vi "50-2.vi"() -> ()   [LabVIEW 2025]
uses:
  <vilib>/Platform/TimedLoop/XDataNode/timing_clust.ctl
  <vilib>/Platform/TimedLoop/XDataNode/nitl_modes.ctl
  <vilib>/Platform/TimedLoop/XDataNode/wakeup.ctl
  <vilib>/eio/utilities/niEioResolveVilibRelativePath.vi
  <vilib>/rvi/interface/RandomDataEmulation/niFpgaRandomDataHandleErrors.vi
  <vilib>/rvi/Memory/Memory_Emulation/nirvimemoryFastEmulation.vi
  <vilib>/rvi/Memory/Memory_Emulation/nirvimemoryEmulation.vi
  <vilib>/rvi/Emulation/niFpgaEmulationIsFPGAContextNoSignature.vi
  <vilib>/rvi/DataTransferAndStorage/Container/Common/niFpgaContainerGetUniqueNameForEmu.vi
  <vilib>/rvi/Emulation/niFpgaProcessEmulError.vi
  <vilib>/rvi/Emulation/niFpgaSctlEmulationGetInTimedLoop.vi
  <vilib>/rvi/errors/nirviReportUnexpectedCaseInternalError (U32).vi
  <vilib>/rvi/Emulation/niFpgaEmulationReportErrorSimple.vi
  <vilib>/rvi/Emulation/niFpgaGetClockAttributes.vi
  <vilib>/rvi/Emulation/niFpgaCriticalErrorInLSC.vi
  <vilib>/rvi/linearAlgebra/MatrixMultiply/simVIs/SubVI/nifxpla_MatrixMultiply_SimMatrixSizes.vi
  <vilib>/rvi/linearAlgebra/MatrixMultiply/simVIs/SubVI/nifxpla_MatrixMultiply_Sim4WireAdapterVector.vi
  <vilib>/rvi/linearAlgebra/MatrixMultiply/simVIs/SubVI/nifxpla_MatrixMultiply_SimFrameHandShake.vi
  <vilib>/rvi/linearAlgebra/MatrixMultiply/simVIs/SubVI/nifxpla_MatrixMultiply_SimEndlessCounter.vi
  <vilib>/rvi/linearAlgebra/MatrixMultiply/simVIs/SubVI/nifxpla_MatrixMultiply_SimVectorDataBuffer.vi
  <vilib>/rvi/ClientSDK/Core/DevComputerLib/Private/Multiply(dfxp64).vi
  <vilib>/rvi/ClientSDK/Core/DevComputerLib/Private/Dfxp128ToDfxp256.vi
  <vilib>/rvi/ClientSDK/Core/DevComputerLib/Private/Add(dfxp256).vi
  <vilib>/rvi/ClientSDK/Core/DevComputerLib/Private/Subtract(dfxp256).vi
  <vilib>/rvi/ClientSDK/Core/DevComputerLib/Private/ToDfxp64(dfxp256).vi
  <vilib>/rvi/DataTransferAndStorage/Container/XNode/niFpgaContainer.xnode
  <vilib>/rvi/interface/RandomDataEmulation/nirviRandomDataFpgaReadWriteTemplate.vi
  <vilib>/platform/TimedLoop/XDataNode/XDataNode.xnode
  <vilib>/rvi/linearAlgebra/MatrixMultiply/XNode/nifxpla_MatrixMultiply.xnode
  <vilib>/rvi/linearAlgebra/MatrixMultiply/simVIs/nifxpla_MatrixMultiply_SimTemplateEinEout.vi
  <vilib>/rvi/linearAlgebra/MatrixMultiply/simVIs/nifxpla_MatrixMultiply_SimTemplateEinVout.vi
  <vilib>/rvi/linearAlgebra/MatrixMultiply/simVIs/nifxpla_MatrixMultiply_SimTemplateVinEout.vi
  <vilib>/rvi/linearAlgebra/MatrixMultiply/simVIs/nifxpla_MatrixMultiply_SimTemplateVinVout.vi
  <vilib>/Platform/TimedLoop/XDataNode/XDNodeRunTimeDep.lvlib
panel:
  out "Latency":u32
  out "Cycle Count":i32
  out "C1":fxp<+/-,32,16>[](array[numeric])
  out "C1+B":fxp<+/-,33,17>[](array[numeric])
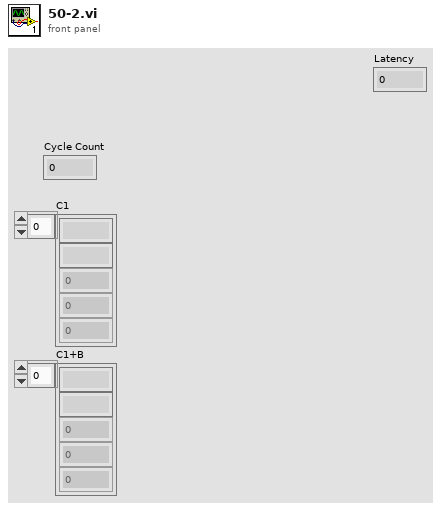
[diagram p1: front panel]
types:
  T1 = typedef "XDNodeRunTimeDep.lvlib/timing_clust.ctl" = cluster{"Expected End [f-1]":u64, "Actual End [f-1]":u64, "Finished Late? [f-1]":bool, "Expected End [i-1]":u64, "Actual End [i-1]":u64, "Finished Late? [i-1]":bool, "Expected Start [i]":u64, "Actual Start [i]":u64, "Expected Start [f]":u64, "Actual Start [f]":u64, "Source Name":string, "Structure Name":string, "Period":i64, "Deadline":i64, "Offset":i64, "Start":i64, "Priority":i32, "Timeout":i32, "Mode":T2, "Wakeup Reason":T3, "Error":errorcluster, "Source Type":string, "Secondary Source Type":string, "Global End Time":u64, "Global Start Time":u64, "Frame Duration":u64, "Iteration Duration":u64, "Assigned CPU":i32, "I/O Scan Engine Mode":u32}
  T2 = typedef "XDNodeRunTimeDep.lvlib/nitl_modes.ctl" = enum32{"No Change", "Process missed periods, maintain original phase", "Discard missed periods, maintain original phase", "Process missed periods, ignore original phase", "Discard missed periods, ignore original phase"}
  T3 = typedef "XDNodeRunTimeDep.lvlib/wakeup.ctl" = enum32{"Normal", "Aborted", "Asynchronous wakeup", "Timing source error", "Timed loop error", "Timeout"}
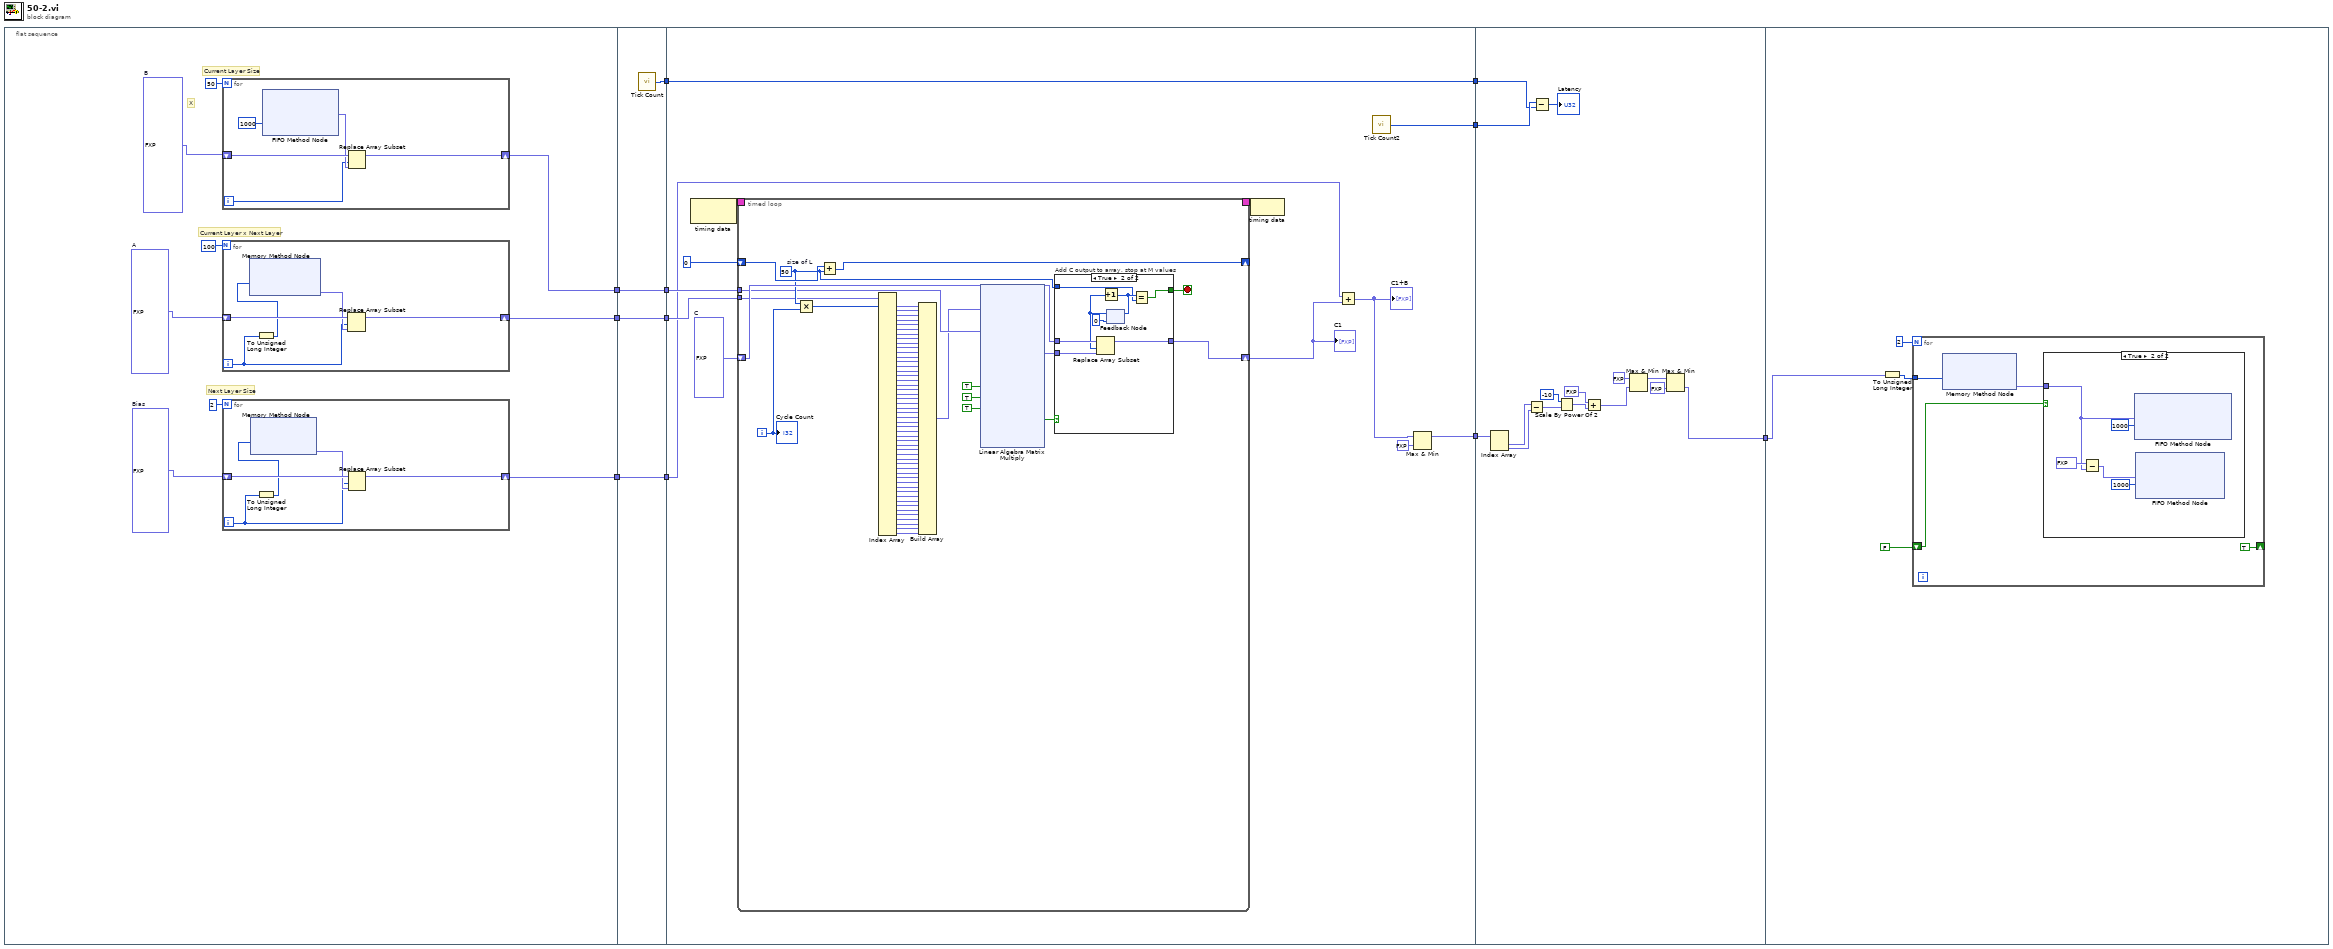
[diagram p0: block diagram]
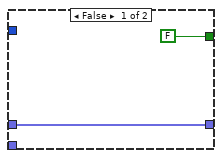
[diagram p2: hidden frame]
diagram:
  n1 = flat-sequence {
    tunnel: [w16] -> w7
    tunnel: [w13] -> w5
    tunnel: [w12] -> w2
    tunnel: [w39] -> w11
    tunnel: [w38] -> w8
    tunnel: w7 -> [w38]
    tunnel: [w37] -> w6
    tunnel: w5 -> [w37]
    tunnel: w2 -> [w36]
    tunnel: [w36] -> w1
    tunnel: [w52] -> w10
    tunnel: [w51] -> w9
    tunnel: [w49] -> w4
    tunnel: w11 -> [w52]
    tunnel: w8 -> [w43]
    tunnel: w6 -> [w40]
    tunnel: w1 -> [w41]
    tunnel: w10 -> [w146]
    tunnel: w9 -> [w147]
    tunnel: w4 -> [w144]
    tunnel: [w133] -> w3
    tunnel: w3 -> [w149]
    frame #0 {
      w14 = fxp<+/-,32,16>[] [0.0, 0.0]  # Bias
      w17 = fxp<+/-,32,16>[] [0.0, 0.0, 0.0, 0.0, 0.0, 0.0, 0.0, 0.0, 0.0, 0.0, 0.0, 0.0, 0.0, 0.0, 0.0, 0.0, 0.0, 0.0, 0.0, 0.0, 0.0, 0.0, 0.0, 0.0, 0.0, 0.0, 0.0, 0.0, 0.0, 0.0, 0.0, 0.0, 0.0, 0.0, 0.0, 0.0, 0.0, 0.0, 0.0, 0.0, 0.0, 0.0, 0.0, 0.0, 0.0, 0.0, 0.0, 0.0, 0.0, 0.0, 0.0, 0.0, 0.0, 0.0, 0.0, 0.0, 0.0, 0.0, 0.0, 0.0, 0.0, 0.0, 0.0, 0.0, 0.0, 0.0, 0.0, 0.0, 0.0, 0.0, 0.0, 0.0, 0.0, 0.0, 0.0, 0.0, 0.0, 0.0, 0.0, 0.0, 0.0, 0.0, 0.0, 0.0, 0.0, 0.0, 0.0, 0.0, 0.0, 0.0, 0.0, 0.0, 0.0, 0.0, 0.0, 0.0, 0.0, 0.0, 0.0, 0.0]  # A
      w19 = fxp<+/-,32,16>[] [0.0, 0.0, 0.0, 0.0, 0.0, 0.0, 0.0, 0.0, 0.0, 0.0, 0.0, 0.0, 0.0, 0.0, 0.0, 0.0, 0.0, 0.0, 0.0, 0.0, 0.0, 0.0, 0.0, 0.0, 0.0, 0.0, 0.0, 0.0, 0.0, 0.0, 0.0, 0.0, 0.0, 0.0, 0.0, 0.0, 0.0, 0.0, 0.0, 0.0, 0.0, 0.0, 0.0, 0.0, 0.0, 0.0, 0.0, 0.0, 0.0, 0.0]  # B
      # "Next Layer Size"
      # "Current Layer Size"
      # "Current Layer x Next Layer"
      # "X"
      n2 = for {
        N: 100 -> [_]
        shift-right: [w29] -> w12
        shift-left: w17 -> [w30]
        i -> [w27]
        n3 = To Unsigned Long Integer(number=w27) -> (unsigned 32bit integer=w26:u32)
        n4 = xnode ("Memory Method Node")("Address"=w26) -> ("Data"=w28:fxp<+/-,32,16>)  [unwired: 1 in, 1 out]
        n5 = Replace Array Subset(array=w30, new element=w28, index=w27) -> (w29:fxp<+/-,32,16>[])
      }
      n6 = for {
        N: 50 -> [_]
        shift-right: [w32] -> w16
        shift-left: w19 -> [w34]
        i -> [w31]
        n7 = xnode ("FIFO Method Node")("Timeout"=1000) -> ("Element"=w33:fxp<+/-,32,16>)  [unwired: 1 in, 2 out]
        n8 = Replace Array Subset(array=w34, new element=w33, index=w31) -> (w32:fxp<+/-,32,16>[])
      }
      n9 = for {
        N: 2 -> [_]
        shift-right: [w24] -> w13
        shift-left: w14 -> [w25]
        i -> [w22]
        n10 = To Unsigned Long Integer(number=w22) -> (unsigned 32bit integer=w21:u32)
        n11 = xnode ("Memory Method Node")("Address"=w21) -> ("Data"=w23:fxp<+/-,32,16>)  [unwired: 1 in, 1 out]
        n12 = Replace Array Subset(array=w25, new element=w23, index=w22) -> (w24:fxp<+/-,32,16>[])
      }
    }
    frame #1 {
      n13 = call "Tick Count"() -> ("Tick Count(Ticks)"=w39:u32)
    }
    frame #2 {
      w46 = fxp<+/-,32,16>[] [0.0, 0.0]  # C
      n14 = node-c288() -> (w48:T1)  [unwired: 1 in]
      n15 = timed-loop {
        timing: w48 -> [_]
        timing-out: [_] -> w47
        shift-right: [w117] -> w44
        shift-left: w46 -> [w116]
        shift-right: [w110] -> _
        shift-left: 0 ("length") -> [w111]
        tunnel: w41 -> [w59]
        tunnel: w43 -> [w58]
        i -> [w97]
        stop <- w115 stop-if-true
        w96 = 50  # size of L
        n16 = Multiply(x=w96, y=w97) -> (x*y=w108:i32)
        n17 = Add(x=w111, y=w96) -> (x+y=w110:i32)
        n18 = Index Array(array=w59, index #1=w108) -> (element #1=w107:fxp<+/-,32,16>, element #2=w106:fxp<+/-,32,16>, element #3=w105:fxp<+/-,32,16>, element #4=w104:fxp<+/-,32,16>, element #5=w103:fxp<+/-,32,16>, element #6=w102:fxp<+/-,32,16>, element #7=w101:fxp<+/-,32,16>, element #8=w100:fxp<+/-,32,16>, element #9=w99:fxp<+/-,32,16>, element #10=w98:fxp<+/-,32,16>, element #11=w95:fxp<+/-,32,16>, element #12=w94:fxp<+/-,32,16>, element #13=w93:fxp<+/-,32,16>, element #14=w92:fxp<+/-,32,16>, element #15=w91:fxp<+/-,32,16>, element #16=w90:fxp<+/-,32,16>, element #17=w89:fxp<+/-,32,16>, element #18=w88:fxp<+/-,32,16>, element #19=w87:fxp<+/-,32,16>, element #20=w86:fxp<+/-,32,16>, element #21=w85:fxp<+/-,32,16>, element #22=w84:fxp<+/-,32,16>, element #23=w83:fxp<+/-,32,16>, element #24=w82:fxp<+/-,32,16>, element #25=w81:fxp<+/-,32,16>, element #26=w80:fxp<+/-,32,16>, element #27=w79:fxp<+/-,32,16>, element #28=w78:fxp<+/-,32,16>, element #29=w77:fxp<+/-,32,16>, element #30=w76:fxp<+/-,32,16>, element #31=w75:fxp<+/-,32,16>, element #32=w74:fxp<+/-,32,16>, element #33=w73:fxp<+/-,32,16>, element #34=w71:fxp<+/-,32,16>, element #35=w72:fxp<+/-,32,16>, element #36=w70:fxp<+/-,32,16>, element #37=w69:fxp<+/-,32,16>, element #38=w68:fxp<+/-,32,16>, element #39=w67:fxp<+/-,32,16>, element #40=w56:fxp<+/-,32,16>, element #41=w66:fxp<+/-,32,16>, element #42=w65:fxp<+/-,32,16>, element #43=w64:fxp<+/-,32,16>, element #44=w63:fxp<+/-,32,16>, element #45=w61:fxp<+/-,32,16>, element #46=w62:fxp<+/-,32,16>, element #47=w60:fxp<+/-,32,16>, element #48=w55:fxp<+/-,32,16>, element #49=w54:fxp<+/-,32,16>, element #50=w53:fxp<+/-,32,16>)  [unwired: 49 in]
        n19 = Build Array(w107, w106, w105, w104, w103, w102, w101, w100, w99, w98, w95, w94, w93, w92, w91, w90, w89, w88, w87, w86, w85, w84, w83, w82, w81, w80, w79, w78, w77, w76, w75, w74, w73, w71, w72, w70, w69, w68, w67, w56, w66, w65, w64, w63, w61, w62, w60, w55, w54, w53) -> (w57:fxp<+/-,32,16>[])
        n20 = xnode ("Linear Algebra Matrix Multiply")("ar"=w57, "br"=w58, "a valid"=TRUE, "b valid"=TRUE, "ready for output (T)"=TRUE) -> ("cr"=w113:fxp<+/-,64,38>[], "output valid"=w109:bool)  [unwired: 2 in, 4 out]
        n21 = case "Add C output to array, stop at M values" shown="True" w109 {
          tunnel: w113 -> [_ w124]
          tunnel: [w120 w127] -> w117
          tunnel: w116 -> [w120 w128]
          tunnel: [FALSE w125] -> w115
          tunnel: w96 -> [_ w121]
          frame False {
          }
          frame True {
            n22 = feedback #1(0 ("x")) -> (w123:i32)
            n23 = Replace Array Subset(array=w128, new element=w124, index=w123) -> (w127:fxp<+/-,32,16>[])
            n24 = Increment(x=w123) -> (x+1=w122:i32)
            n25 = feedback-in #1(w122) -> ()
            n26 = Equal?(x=w122, y=w121) -> (x = y?=w125:bool)
          }
        }
        "Cycle Count" <- w97
      }
      "C1" <- w44
      n27 = node-c288(w47) -> ()
      n28 = Add(x=w40, y=w44) -> (x+y=w42:fxp<+/-,33,17>[])
      "C1+B" <- w42
      n29 = call "Tick Count2"() -> ("Tick Count(Ticks)"=w51:u32)
      n30 = Max & Min(x=w42, y=fxp<+,1,1> 0.0) -> (max(x,y)=w49:fxp<+/-,33,17>[])  [unwired: 1 out]
    }
    frame #3 {
      n31 = Index Array(array=w144) -> (element #1=w135:fxp<+/-,33,17>, element #2=w134:fxp<+/-,33,17>)  [unwired: 2 in]
      n32 = Subtract(x=w135, y=w134) -> (x-y=w140:fxp<+/-,34,18>)
      n33 = Subtract(x=w147, y=w146) -> (x-y=→"Latency":u32)
      n34 = Scale By Power Of 2(n=i16 -10, x=w140) -> (x*2^n=w141:fxp<+/-,34,18>)
      n35 = Add(x=fxp<+,1,9> 256.0, y=w141) -> (x+y=w142:fxp<+/-,35,19>)
      n36 = Max & Min(x=fxp<+,1,1> 0.0, y=w142) -> (max(x,y)=w143:fxp<+/-,35,19>)  [unwired: 1 out]
      n37 = Max & Min(x=w143, y=fxp<+,9,9> 511.0) -> (min(x,y)=w133:fxp<+/-,35,19>)  [unwired: 1 out]
    }
    frame #4 {
      n38 = To Unsigned Long Integer(number=w149) -> (unsigned 32bit integer=w148:u32)
      n39 = for {
        N: 2 -> [_]
        tunnel: w148 -> [w155]
        shift-right: [TRUE] -> _
        shift-left: FALSE -> [w154]
        n40 = xnode ("Memory Method Node")("Address"=w155) -> ("Data"=w152:fxp<+/-,32,16>)  [unwired: 1 in, 1 out]
        n41 = case shown="True" w154 {
          tunnel: w152 -> [_ w156]
          frame False {
          }
          frame True {
            n42 = Subtract(x=fxp<+,1,16> 32768.0, y=w156) -> (x-y=w160:fxp<+,33,17>)
            n43 = xnode ("FIFO Method Node")("Element"=w156, "Timeout"=1000) -> ()  [unwired: 1 in, 2 out]
            n44 = xnode ("FIFO Method Node")("Element"=w160, "Timeout"=1000) -> ()  [unwired: 1 in, 2 out]
          }
        }
      }
    }
  }
